vi "_Subsystem_Name Global.vi"() -> ()   [LabVIEW 2023]
uses:
  Drive Conditions.ctl
panel:
  in  "Drive Conditions":T1
  in  "Max Drive Speed":dbl=17.49
  # "This is one place you may want to put\ntuning and debugging parameters."
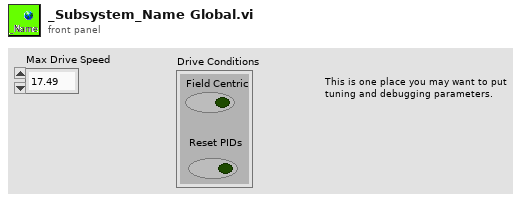
[diagram p1: front panel]
types:
  T1 = typedef "Drive Conditions.ctl" = cluster{"Field Centric":bool, "Reset PIDs":bool}
diagram:
